vi "Set Logger Enqueuer.vi"(8 "error in":errorcluster, 10 "Logger":refnum<class "Message Enqueuer.lvclass">, 11 "ILogger Client in":refnum<class "ILogger Client.lvclass">) -> (0 "error out":errorcluster, 3 "ILogger Client out":refnum<class "ILogger Client.lvclass">)   [LabVIEW 2026, in "ILogger Client.lvlib" / "ILogger Client.lvclass"]
doc: "Set the logger enqueuer for a Logger Client."
uses:
  ILogger Client.lvclass
  <vilib>/ActorFramework/Message Enqueuer/Message Enqueuer.lvclass
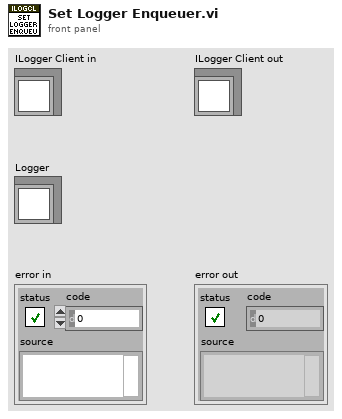
[diagram p1: front panel]
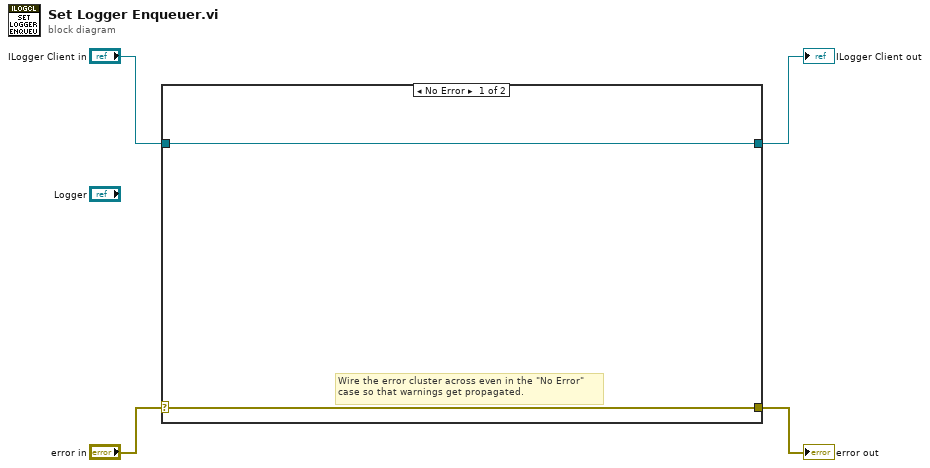
[diagram p0: block diagram]
diagram:
  n1 = case shown="No Error" "error in" {
    selector: "error in" -> [w6 w8]
    tunnel: [w6 w8] -> w3
    tunnel: [w5 w7] -> w1
    tunnel: "ILogger Client in" -> [w5 w7]
    frame No Error {
      # "Wire the error cluster across even in the \"No Error\"\ncase so that warnings get propagated."
    }
    frame Error {
    }
  }
  "error out" <- w3
  "ILogger Client out" <- w1
